vi "Stress_Calc_SubVI.vi"(0 "current":dbl, 1 "temp":dbl, 2 "tar curr":dbl, 3 "max temp lim":dbl) -> (4 "stress inx":dbl, 5 "throttled  curr":dbl, 6 "ctrl vol":dbl)   [LabVIEW 2019]
panel:
  in  "voltage":dbl
  # "INPUT"
  # "OUTPUT"
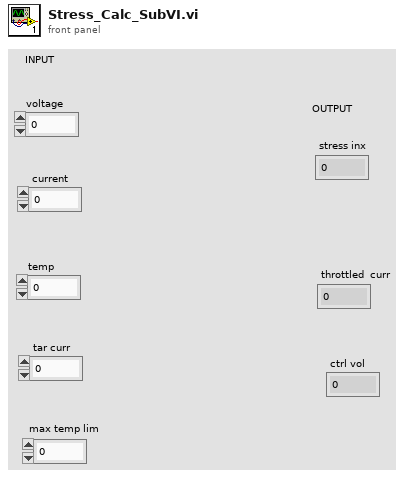
[diagram p1: front panel]
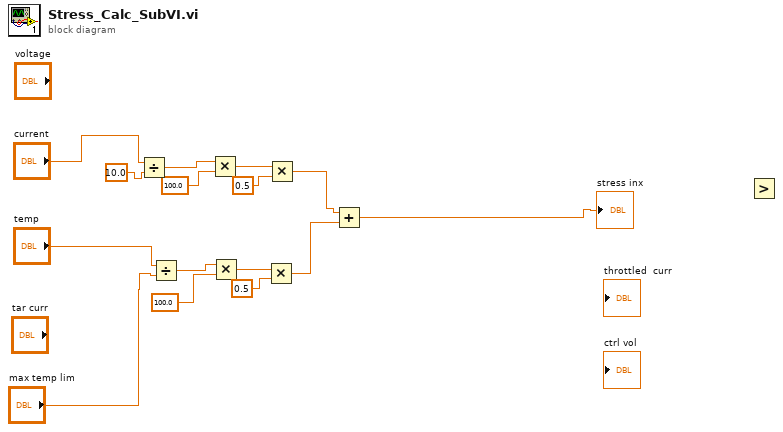
[diagram p0: block diagram]
diagram:
  n1 = Divide(x="current", y=10.0) -> (x/y=w9:dbl)
  n2 = Divide(x="temp", y="max temp lim") -> (x/y=w13:dbl)
  n3 = Multiply(x=w9, y=100.0) -> (x*y=w7:dbl)
  n4 = Multiply(x=w13, y=100.0) -> (x*y=w5:dbl)
  n5 = Multiply(x=w5, y=0.5) -> (x*y=w2:dbl)
  n6 = Multiply(x=w7, y=0.5 ("x*y")) -> (x*y=w3:dbl)
  n7 = Add(x=w3, y=w2) -> (x+y=→"stress inx":dbl)
  n8 = Greater?() -> ()  [unwired: 2 in, 1 out]
